vi "When Call Function.vi"(0 "error out":errorcluster, 2 "Return String":string, 11 "IPython Caller in":refnum<class "Mock IPython Caller.lvclass">) -> (3 "IPython Caller out":refnum<class "Mock IPython Caller.lvclass">)   [LabVIEW 2026, in "Mock IPython Caller.lvclass"]
doc: "This VI calls the specified function from a python script. This VI can only call functions with a string input and output parameter. The function uses the tool global virtual environment."
uses:
  Mock IPython Caller.lvclass
  Mock IPython Caller.lvclass/Mock IPython Caller.ctl
  C:/Program Files/National Instruments/LabVIEW 2026/vi.lib/Astemes/LMock/Mock.lvclass
  C:/Users/juanj/Documents/hasbun_wood_engineering/github/py2vi/labview/Mocks/Mock IPython Caller/Mock IPython Caller.lvclass
  C:/Users/juanj/Documents/hasbun_wood_engineering/github/py2vi/labview/Interfaces/IPython Caller/IPython Caller.lvclass
  <vilib>/Astemes/LMock/Mock.lvclass
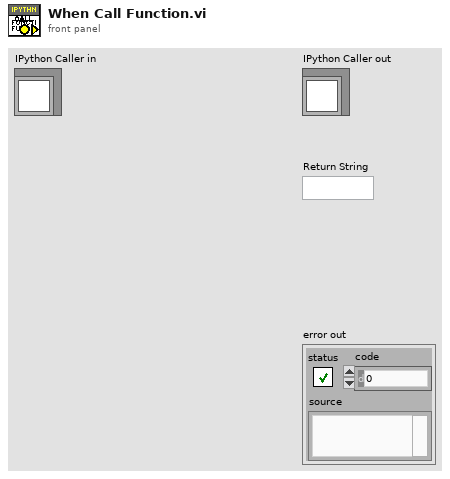
[diagram p1: front panel]
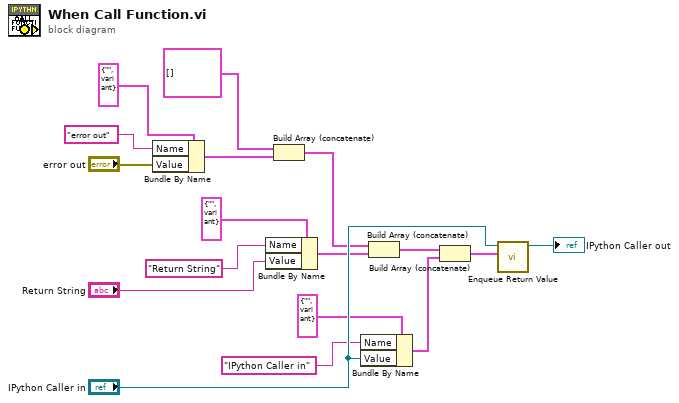
[diagram p0: block diagram]
diagram:
  n1 = Bundle By Name(cluster=cluster{"Name":string, "Value":variant} {"Name"="", "Value"=variant} ("element"), "Name"="error out", "Value"="error out") -> (w5:cluster{"Name":string, "Value":variant})
  n2 = Bundle By Name(cluster=cluster{"Name":string, "Value":variant} {"Name"="", "Value"=variant} ("element"), "Name"="Return String", "Value"="Return String") -> (w3:cluster{"Name":string, "Value":variant})
  n3 = Build Array (concatenate)(cluster{"Name":string, "Value":variant}[] [] ("Control Values"), w5) -> (w10:cluster{"Name":string, "Value":variant}[])
  n4 = Bundle By Name(cluster=cluster{"Name":string, "Value":variant} {"Name"="", "Value"=variant} ("element"), "Name"="IPython Caller in", "Value"="IPython Caller in") -> (w1:cluster{"Name":string, "Value":variant})
  n5 = Build Array (concatenate)(w10, w3) -> (w13:cluster{"Name":string, "Value":variant}[])
  n6 = Build Array (concatenate)(w13, w1) -> (w15:cluster{"Name":string, "Value":variant}[])
  n7 = call <vilib>:"Enqueue Return Value.vi"("Indicator Values"=w15, "Mock In"="IPython Caller in") -> ("Mock Out"=→"IPython Caller out":refnum<class "Mock IPython Caller.lvclass">)  [unwired: 8 in, 1 out]
